vi "Identify and Replace Entire Element.vi"(7 "Named Cluster":variant, 8 "Identifying Attribute Value":string, 9 "Identifying Attribute Type":string, 10 "Element Type":string, 11 "XML String":string) -> (3 "Edited XML":string)   [LabVIEW 2019, in "EditSVG.lvclass"]
uses:
  EditSVG.lvclass
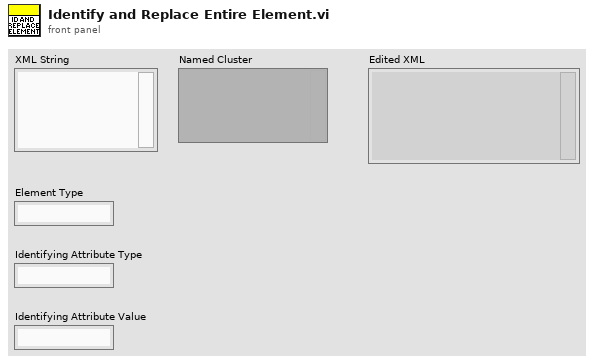
[diagram p1: front panel]
types:
  T1 = cluster{"width":string, "height":string, "preserveAspectRatio":string, "xlink:href":string, "id":string, "x":string, "y":string}
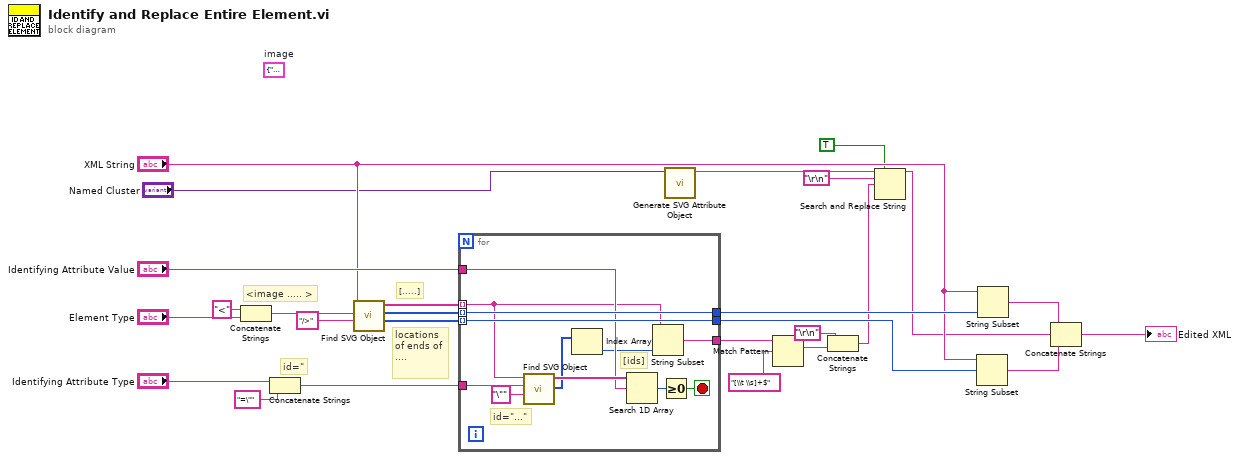
[diagram p0: block diagram]
diagram:
  (unwired) T1 {"width"="250", "height"="500", "preserveAspectRatio"="none", "xlink:href"="Mock%20Device2.jpg", "id"="image1-4-5-1", "x"="222", "y"="551"}  # image
  # "id=\""
  # "locations of ends of ...."
  # "[.....]"
  # "<image ..... >"
  n1 = Concatenate Strings("<" ("string"), "Element Type") -> (w21:string)
  n2 = Concatenate Strings("Identifying Attribute Type", "=\"" ("string")) -> (w24:string)
  n3 = call "Find SVG Object.vi"("Ending Delimiter"="/>", "Beginning Delimiter"=w21, "XML String"="XML String") -> ("Ending Indices"=w23:i32[], "Beginning Indices"=w17:i32[], "Found Values"=w26:string[])  [unwired: 6 in]
  n4 = for {
    tunnel: w26 -> [w28] mode=indexing
    tunnel: w24 -> [w38]
    tunnel: "Identifying Attribute Value" -> [w31]
    tunnel: w23 -> [w37] mode=indexing
    tunnel: [w37] -> w15
    tunnel: [w33] -> w16
    tunnel: w17 -> [w33] mode=indexing
    tunnel: [w29] -> w10
    stop <- w34 stop-if-true
    # "id=\"...\""
    # "[ids]"
    n5 = call "Find SVG Object.vi"("Ending Delimiter"="\"", "Beginning Delimiter"=w38, "XML String"=w28) -> ("Beginning Indices"=w32:i32[], "Found Values"=w36:string[])  [unwired: 6 in, 1 out]
    n6 = Index Array(array=w32) -> (element=w30:i32)  [unwired: 1 in]
    n7 = Search 1D Array(1D array=w36, element=w31) -> (index of element=w35:i32)  [unwired: 1 in]
    n8 = String Subset(string=w28, length (rest)=w30) -> (substring=w29:string)  [unwired: 1 in]
    n9 = Greater Or Equal To 0?(x=w35) -> (x >= 0?=w34:bool)
  }
  n10 = call "Generate SVG Attribute Object.vi"("Named Cluster of Data"="Named Cluster") -> ("SVG Attribute Object"=w9:string)  [unwired: 9 in, 1 out]
  n11 = Match Pattern(string=w10, regular expression="[\\t \\s]+$") -> (match substring=w4:string)  [unwired: 1 in, 3 out]
  n12 = Concatenate Strings("\r\n", w4) -> (w3:string)
  n13 = Search and Replace String(replace all?=TRUE ("replace all? (F)"), input string=w9, search string="\r\n", replace string=w3) -> (result string=w8:string)  [unwired: 4 in, 3 out]
  n14 = String Subset(string="XML String", offset (0)=w15) -> (substring=w12:string)  [unwired: 1 in]
  n15 = String Subset(string="XML String", length (rest)=w16) -> (substring=w13:string)  [unwired: 1 in]
  n16 = Concatenate Strings(w13, w8, w12) -> (→"Edited XML":string)
